vi "Convert Press. Sens. V to mmHg.vi"(11 "Waveform":dbl) -> (3 "Numeric":dbl)   [LabVIEW 2024]
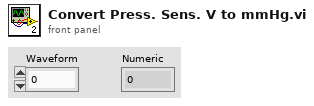
[diagram p1: front panel]
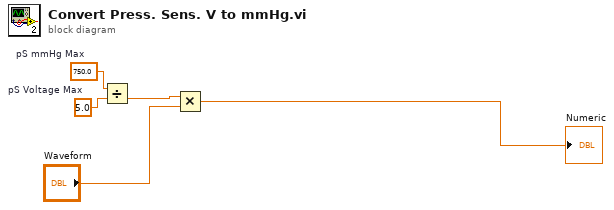
[diagram p0: block diagram]
diagram:
  w3 = 5.0  # pS Voltage Max
  w2 = 750.0  # pS mmHg Max
  n1 = Divide(x=w2, y=w3) -> (x/y=w5:dbl)
  n2 = Multiply(x=w5, y="Waveform") -> (x*y=→"Numeric":dbl)
